vi "Test CTL class.vi"   [LabVIEW 2012]
uses:
  ctl_class/Templates List.ctl
  ctl_class/ctl.lvclass
types:
  T1 = typedef "ctl.lvclass/Templates List.ctl" = enum16{"System", "Vista 54 x 54 ", "user-defined"}
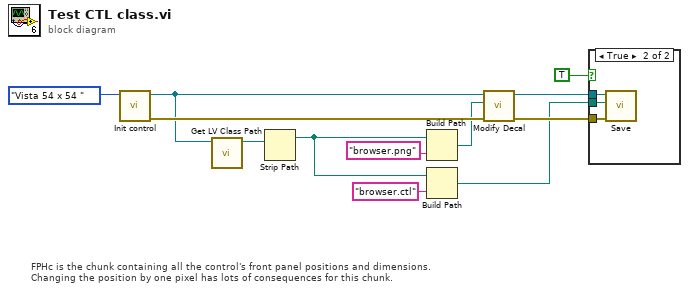
[diagram p0: block diagram]
diagram:
  # "FPHc is the chunk containing all the control's front panel positions and dimensions.\nChanging the position by one pixel has lots of consequences for this chunk."
  n1 = call "Init control.vi"("Template (System)"=Templates_List."Vista 54 x 54 ") -> ("error out"=w12:errorcluster, "ctl out"=w6:refnum<class "ctl.lvclass">)  [unwired: 3 in, 6 out]
  n2 = call <vilib>:"Get LV Class Path.vi"("object"=w6) -> ("class path"=w8:path)  [unwired: 1 in, 9 out]
  n3 = Strip Path(path=w8) -> (stripped path=w3:path)  [unwired: 1 out]
  n4 = Build Path(base path=w3, name or relative path="browser.png") -> (appended path=w2:path)
  n5 = Build Path(base path=w3, name or relative path="browser.ctl") -> (appended path=w5:path)
  n6 = call-dynamic "Modify Decal.vi"("error in (no error)"=w12, "new decal"=w2, "ctl in"=w6) -> ("error out"=w9:errorcluster, "ctl out"=w10:refnum<class "ctl.lvclass">)  [unwired: 7 out]
  n7 = case shown="True" TRUE {
    tunnel: w10 -> [_ w15]
    tunnel: w9 -> [_ w14]
    tunnel: w5 -> [_ w13]
    frame False {
    }
    frame True {
      n8 = call-dynamic "Save.vi"("error in (no error)"=w14, "Control path"=w13, "ctl in"=w15) -> ()  [unwired: 9 out]
    }
  }
